vi "HandleItemActivation.vi"(8 "error in (no error)":errorcluster, 11 "Feed_link in":refnum<class "Feed_link.lvclass">) -> (0 "error out":errorcluster, 3 "Feed_link out":refnum<class "Feed_link.lvclass">)   [LabVIEW 2023, in "GettingStartedWindow.lvlib" / "Feed_link.lvclass"]
uses:
  <resource>/modes/FRC/GSW/Classes/Feed_link/Feed_link.lvclass
  home/systemcore/natinst/lvaddons/wpilib/1/resource/modes/FRC/GSW/Classes/Link/Link.lvclass
  <resource>/modes/FRC/GSW/Classes/Feed_link/Feed_link.lvclass/Feed_link.ctl
  <vilib>/NI_RSS/Feed/Feed.lvclass
  <vilib>/Platform/browser.llb/Open URL in Default Browser (string).vi
  <resource>/modes/FRC/GSW/Classes/Link/Link.lvclass
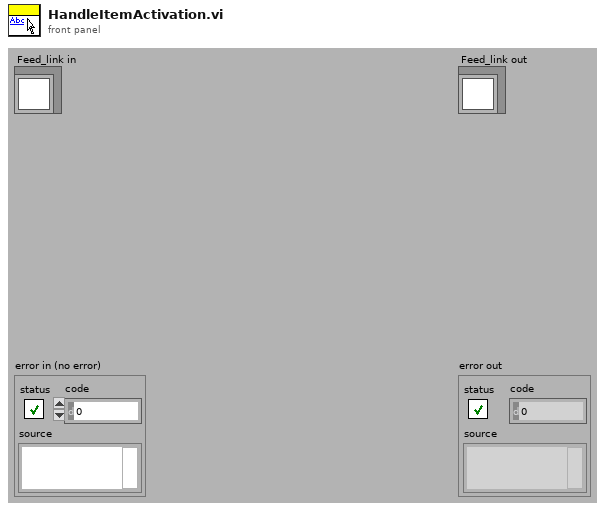
[diagram p1: front panel]
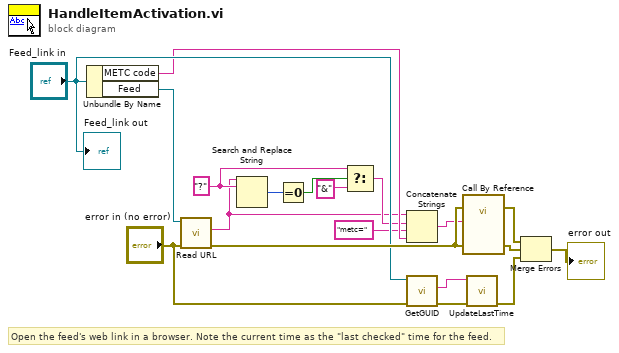
[diagram p0: block diagram]
diagram:
  w5 = "?" ("search string")
  # "Open the feed's web link in a browser. Note the current time as the \"last checked\" time for the feed."
  n1 = Unbundle By Name("Feed_link in") -> ("METC code"=w8:string, "Feed"=w19:refnum<class "Feed.lvclass">)
  n2 = call-dynamic "Read URL.vi"("error in (no error)"="error in (no error)", "Feed.lvclass in"=w19) -> ("error out"=w18:errorcluster, "URL"=w1:string)  [unwired: 8 out]
  n3 = Search and Replace String(input string=w1, search string=w5) -> (number of replacements=w7:i32)  [unwired: 1 in, 8 out]
  n4 = Equal To 0?(x=w7) -> (x = 0?=w6:bool)
  n5 = Select(t=w5, s=w6, f="&") -> (s? t:f=w2:string)
  n6 = Concatenate Strings(w1, w2, "metc=" ("format string"), w8) -> (w9:string)
  n7 = call <resource>:"GetGUID.vi"("error in (no error)"="error in (no error)", "Link in"="Feed_link in") -> ("error out"=w15:errorcluster, "GUID"=w16:string)  [unwired: 8 out]
  n8 = call-by-ref "?"(error in=w18, 4:"error in (no error)"=w18, "URL"=w9) -> (error out=w13:errorcluster, 0:"error out"=w12:errorcluster)  [unwired: 1 in, 6 out]
  n9 = call <resource>:"UpdateLastTime.vi"("error in (no error)"=w15, "feed GUID"=w16) -> ("error out"=w11:errorcluster)  [unwired: 9 out]
  n10 = Merge Errors(w13, w12, w11) -> (→"error out":errorcluster)
  "Feed_link out" <- "Feed_link in"
